vi "Step_Cancel.vi"(8 "error in (no error)":errorcluster={"status"=FALSE, "code"=0, "source"="\"\""}, 10 "stop/fault reason":string, 11 "StepContext":string) -> (0 "error out":errorcluster={"status"=FALSE, "code"=0, "source"="\"\""}, 2 "status ok":bool, 3 "Cancelled status":string)   [LabVIEW 2026]
doc: "INTENT: Cancel action and cleanup. LOGIC: Cancel capture, plugin request and outstanding commands; release leases; mark partial results."
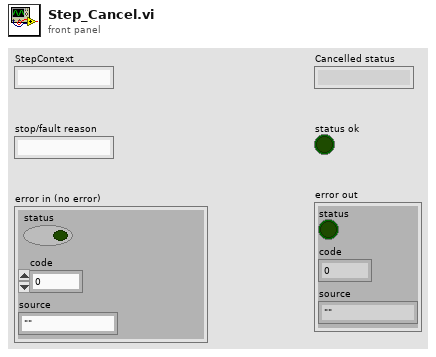
[diagram p1: front panel]
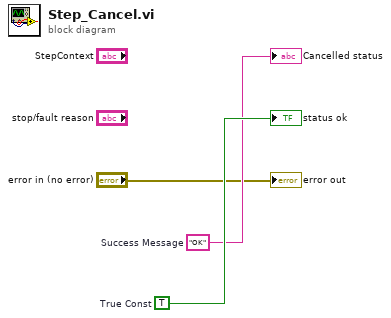
[diagram p0: block diagram]
diagram:
  w3 = TRUE  # True Const
  w2 = "OK"  # Success Message
  "Cancelled status" <- w2
  "status ok" <- w3
  "error out" <- "error in (no error)"
